vi "Read(Variant).vi"(6 "prioritize Cache? (F)":bool, 7 "Qualified Name":string, 8 "error in (no error)":errorcluster, 9 "Name (empty: type name)":string, 10 "Type":variant, 11 "ConfigManager in":refnum<class "ConfigManager.lvclass">) -> (0 "error out":errorcluster, 2 "value":variant, 3 "ConfigManager out":refnum<class "ConfigManager.lvclass">, 4 "all found?":bool, 5 "any found?":bool)   [LabVIEW 2013, in "CfgManager.lvlib" / "ConfigManager.lvclass"]
uses:
  ConfigManager.lvclass
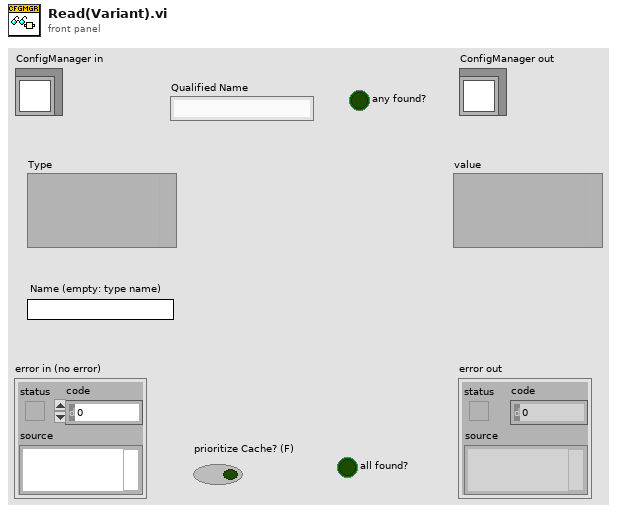
[diagram p1: front panel]
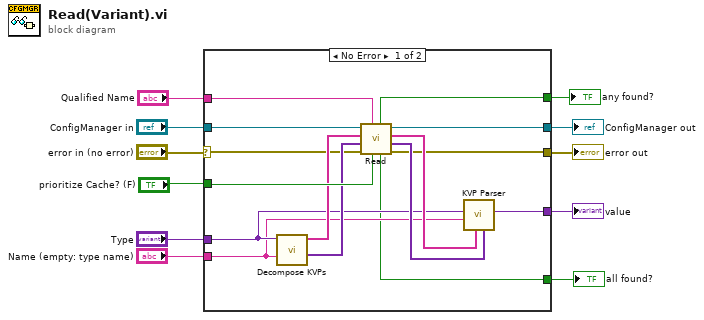
[diagram p0: block diagram]
diagram:
  n1 = case shown="No Error" "error in (no error)" {
    selector: "error in (no error)" -> [w17 w29]
    tunnel: [w16 w29] -> w10
    tunnel: [w15 w28] -> w8
    tunnel: "ConfigManager in" -> [w26 w28]
    tunnel: "Name (empty: type name)" -> [w18 _]
    tunnel: "Type" -> [w19 w27]
    tunnel: [w14 w27] -> w5
    tunnel: "Qualified Name" -> [w25 _]
    tunnel: "prioritize Cache? (F)" -> [w24 _]
    tunnel: [w12 _] -> w2
    tunnel: [w13 _] -> w1
    frame No Error {
      n2 = call "Decompose KVPs.vi"("Name (empty: value name)"=w18, "value"=w19) -> ("Values"=w22:variant[], "Keys"=w23:string[])  [unwired: 8 in]
      n3 = call "Read.vi"("prioritize Cache? (F)"=w24, "Qualified Name"=w25, "error in (no error)"=w17, "Default Values"=w22, "keys in"=w23, "ConfigManager in"=w26) -> ("error out"=w16:errorcluster, "Values"=w20:variant[], "keys"=w21:string[], "ConfigManager out"=w15:refnum<class "ConfigManager.lvclass">, "All Found?"=w13:bool, "Any Found?"=w12:bool)
      n4 = call <vilib>:"KVP Parser.vi"("Values"=w20, "Keys"=w21, "Default Value Name (empty: label)"=w18, "Default Value"=w19) -> ("Value"=w14:variant)  [unwired: 4 in, 3 out]
    }
    frame Error {
    }
  }
  "error out" <- w10
  "ConfigManager out" <- w8
  "value" <- w5
  "any found?" <- w2
  "all found?" <- w1
